vi "Get Language Information.vi"(8 "error in (no error)":errorcluster) -> (0 "error out":errorcluster, 1 "Languages":string[](array[string]), 2 "Default Language":i32, 3 "Start up Language":i32)   [LabVIEW 2019, in "Language Selection.lvlib"]
doc: "Retrieve language settings and defined languages for the translation.\n- - -\nCopyright (c) 2026, Merecs Engineering GmbH"
uses:
  Language Selection.lvlib
panel:
  # "Connector Pane"
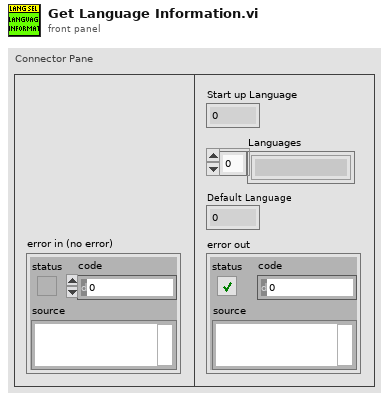
[diagram p1: front panel]
types:
  T1 = typedef "Language Selection.lvlib/Enum Language.ctl" = i32
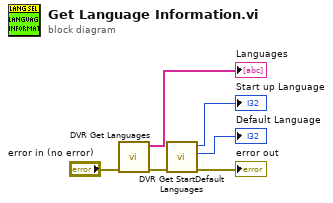
[diagram p0: block diagram]
diagram:
  n1 = call "DVR Get Languages.vi"("error in (no error)"="error in (no error)") -> ("error out"=w2:errorcluster, "Languages"=→"Languages":string[])  [unwired: 7 in, 2 out]
  n2 = call "DVR Get StartDefault Languages.vi"("error in (no error)"=w2) -> ("error out"=→"error out":errorcluster, "Default"=→"Default Language":i32, "Start"=→"Start up Language":T1)  [unwired: 8 in]
